vi "set TXP Sweep Time.vi"(8 "error in (no error)":errorcluster, 10 "Sweep Time(sec)":dbl, 11 "Keysight 9020A in":refnum<class "Keysight 9020A.lvclass">) -> (0 "error out":errorcluster, 3 "Keysight 9020A out":refnum<class "Keysight 9020A.lvclass">)   [LabVIEW 2023, in "Spectrum Analyzer.lvlib" / "Keysight 9020A.lvclass"]
uses:
  Keysight 9020A.lvclass
  Keysight 9020A.lvclass/Keysight 9020A.ctl
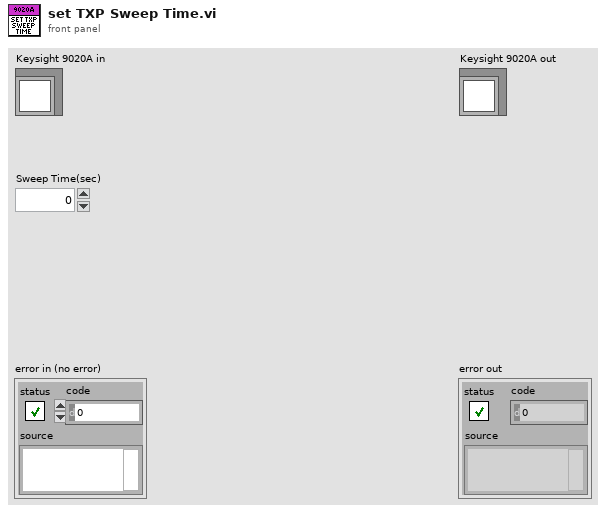
[diagram p1: front panel]
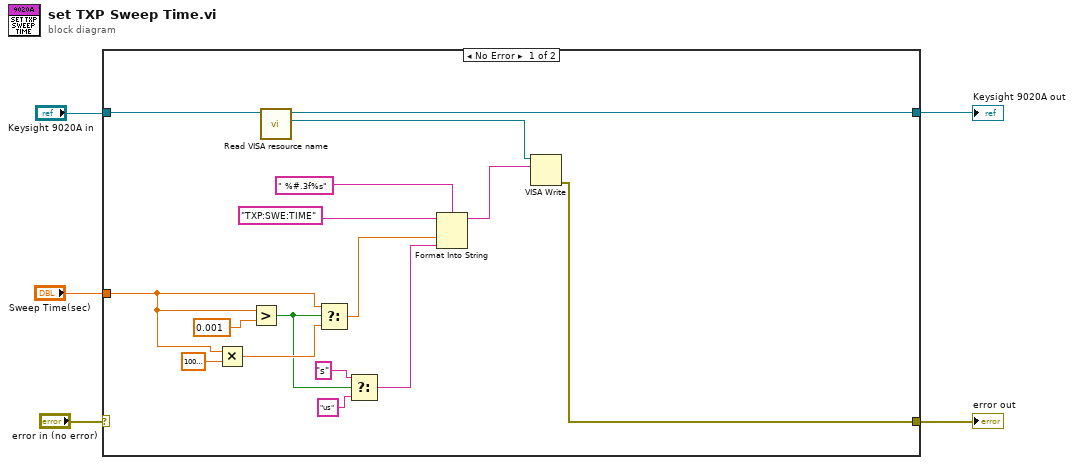
[diagram p0: block diagram]
diagram:
  n1 = case shown="No Error" "error in (no error)" {
    selector: "error in (no error)" -> [_ w22]
    tunnel: "Keysight 9020A in" -> [w17 w23]
    tunnel: [w21 w23] -> w4
    tunnel: [w6 w22] -> w1
    tunnel: "Sweep Time(sec)" -> [w14 _]
    frame No Error {
      n2 = Multiply(x=w14, y=1000000.0) -> (x*y=w13:dbl)
      n3 = Greater?(x=w14, y=0.001) -> (0:w10:bool)
      n4 = call "Read VISA resource name.vi"("Keysight 9020A in"=w17) -> ("VISA resource name"=w18:refnum<visa-resource-name>, "Keysight 9020A out"=w21:refnum<class "Keysight 9020A.lvclass">)  [unwired: 8 in, 1 out]
      n5 = Select(t=w14, s=w10, f=w13) -> (s? t:f=w11:dbl)
      n6 = Select(t="s", s=w10, f="us") -> (s? t:f=w7:string)
      n7 = Format Into String(format string=" %#.3f%s", initial string="TXP:SWE:TIME" ("string"), w11, w7) -> (resulting string=w20:string)  [unwired: 1 in, 1 out]
      n8 = VISA Write(VISA resource name=w18, write buffer=w20) -> (error out=w6:errorcluster)  [unwired: 1 in, 2 out]
    }
    frame Error {
    }
  }
  "error out" <- w1
  "Keysight 9020A out" <- w4
